vi "drawTempRectangle.vi"(0 "reference":refnum<class "Graphics.lvclass">, 1 "rectangle":T1 {"height" format="%.2f"; "width" format="%.2f"; "y" format="%.2f"; "x" format="%.2f"}, 2 "lineWidth(1)":dbl=1.0 format="%.2f", 3 "color(if not used=default color)":u32=33554432 format="%.0x", 4 "fill?(F)":bool, 5 "error in (no error)":errorcluster, 6 "Rectangles":T1[](array[typedef]) {"height" format="%.2f"; "width" format="%.2f"; "y" format="%.2f"; "x" format="%.2f"}, 7 "readFromMaster(True)":bool=TRUE) -> (14 "reference out":refnum<class "Graphics.lvclass">, 16 "picture":picture, 19 "error out":errorcluster)   [LabVIEW 2020, in "Graphics.lvclass"]
doc: "Draws a rectangle"
uses:
  <resource>/Framework/Providers/Open_GDS/UML/Graphics_class/Graphics.lvclass
  <resource>/Framework/Providers/Open_GDS/UML/General/Rectangle/Rectangle Rectangle2D.ctl
panel:
  # "Always set\nVI Server class\nto current VI. Do not\nconnect this control\nto the connector pane.\n(Tip!: Just drag\nand drop the icon\ninto the refnum)"
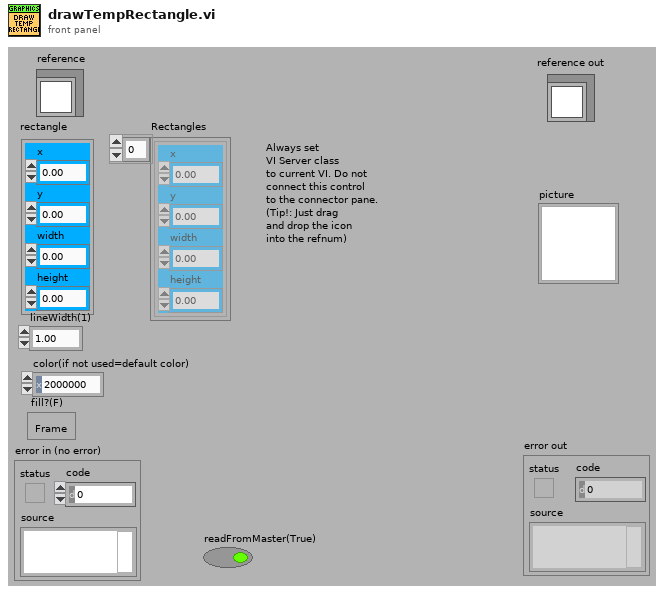
[diagram p1: front panel]
types:
  T1 = typedef "Rectangle Rectangle2D.ctl" = cluster{"x":dbl, "y":dbl, "width":dbl, "height":dbl}
  T2 = typedef "Graphics.lvclass/ObjectAttributes.ctl" = cluster{"drawColor":u32, "backgroundColor":u32, "font":T3, "fontType":T4, "picture":picture, "stroke":T5, "scaleX":dbl, "scaleY":dbl, "screenRef":refnum<vi>, "offsetX":dbl, "offsetY":dbl}
  T3 = typedef "Graphics.lvclass/FontType.ctl" = cluster{"Font Name:":string, "Size":i16, "Strikeout?":bool, "Italic?":bool, "Underline?":bool, "Outline?":bool, "Shadow?":bool, "Bold?":bool}
  T4 = typedef "Graphics.lvclass/LvFontType.ctl" = enum16{"User-specified Font", "Application Font", "System Font", "Dialog Font"}
  T5 = typedef "Graphics.lvclass/StrokeType.ctl" = enum16{"USE_DEFAULT", "SOLID", "DOTTED"}
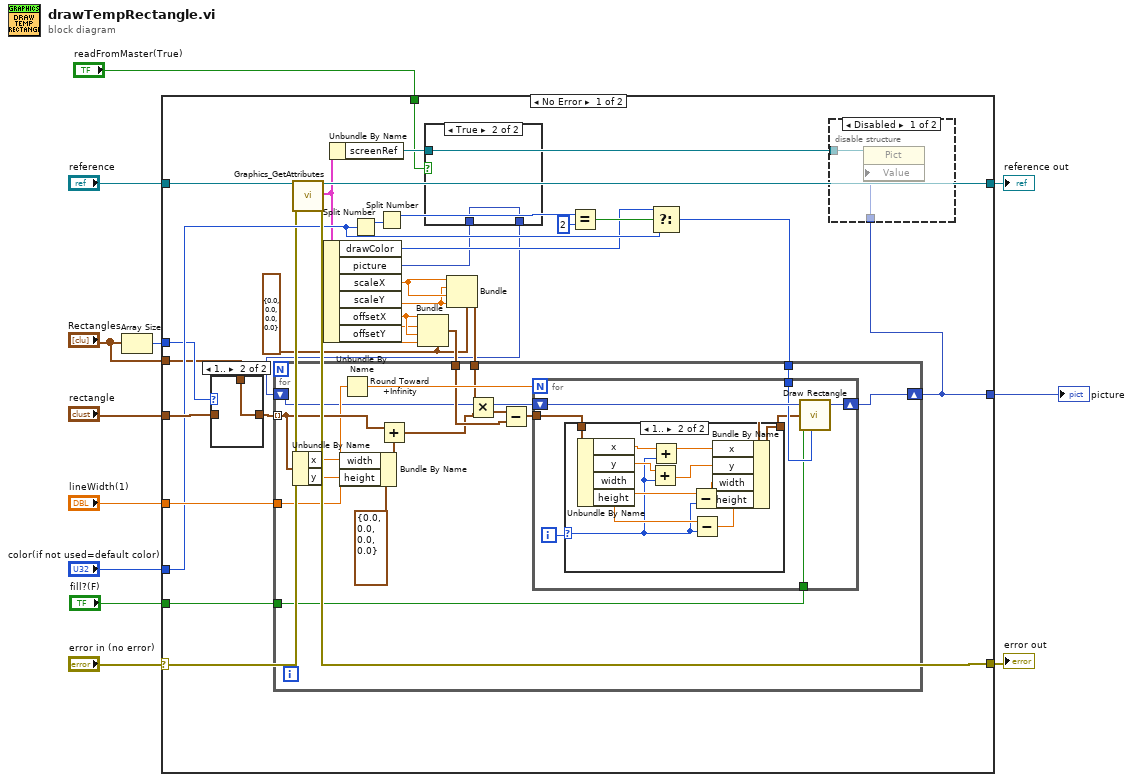
[diagram p0: block diagram]
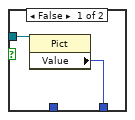
[diagram p3: hidden frame]
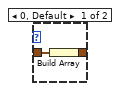
[diagram p4: hidden frame]
diagram:
  n1 = Array Size(array="Rectangles") -> (size(s)=w4:i32)
  n2 = case shown="No Error" "error in (no error)" {
    selector: "error in (no error)" -> [w35 w86]
    tunnel: "reference" -> [w42 w87]
    tunnel: [w41 w86] -> w11
    tunnel: [w40 w87] -> w10
    tunnel: "rectangle" -> [w39 _]
    tunnel: "lineWidth(1)" -> [w38 _]
    tunnel: "color(if not used=default color)" -> [w37 _]
    tunnel: "fill?(F)" -> [w36 _]
    tunnel: w4 -> [w18 _]
    tunnel: "Rectangles" -> [w17 _]
    tunnel: "readFromMaster(True)" -> [w14 _]
    tunnel: [w13 _] -> w1
    frame No Error {
      w20 = T1 {"x"=0.0, "y"=0.0, "width"=0.0, "height"=0.0} ("rectangle")
      n3 = case shown="1.." w18 {
        tunnel: w39 -> [w49 _]
        tunnel: [w48 w50] -> w19
        tunnel: w17 -> [_ w50]
        frame 0, Default {
          n4 = Build Array(w49) -> (w48:T1[])
        }
        frame 1.. {
        }
      }
      n5 = call <resource>:"Graphics_GetAttributes.vi"("reference in"=w42, "error in (no error)"=w35) -> ("reference out"=w40:refnum<class "Graphics.lvclass">, "Data"=w15:T2, "error out"=w41:errorcluster)  [unwired: 1 in, 14 out]
      n6 = Unbundle By Name(w15) -> ("drawColor"=w30:u32, "picture"=w21:picture, "scaleX"=w27:dbl, "scaleY"=w26:dbl, "offsetX"=w25:dbl, "offsetY"=w24:dbl)
      n7 = Unbundle By Name(w15) -> ("screenRef"=w22:refnum<vi>)
      n8 = Split Number(x=w37) -> (hi(x)=w34:u16)  [unwired: 1 out]
      n9 = Split Number(x=w34) -> (hi(x)=w33:u8)  [unwired: 1 out]
      n10 = Bundle(cluster=w20, "x"=w25, "y"=w24, "width"=w25, "height"=w24) -> (w23:T1)
      n11 = case shown="True" w14 {
        tunnel: w22 -> [w46 _]
        tunnel: w21 -> [_ w47]
        tunnel: [w45 w47] -> w16
        frame False {
          n12 = property class="Pict"(reference=w46) -> ("Value"=w45:picture)  [unwired: 1 in, 2 out]
        }
        frame True {
        }
      }
      n13 = Bundle(cluster=w20, "x"=w27, "y"=w26, "width"=w27, "height"=w26) -> (w28:T1)
      n14 = Equal?(x=w33, y=u8 2) -> (x = y?=w31:bool)
      n15 = Select(t=w30, s=w31, f=w37) -> (s? t:f=w29:u32)
      n16 = for {
        tunnel: w19 -> [w66] mode=indexing
        tunnel: w38 -> [w65]
        tunnel: w36 -> [w64]
        tunnel: w29 -> [w62]
        tunnel: w28 -> [w61]
        tunnel: w23 -> [w54]
        shift-right: [w52] -> w13
        shift-left: w16 -> [w51]
        n17 = Unbundle By Name(w66) -> ("x"=w59:dbl, "y"=w58:dbl)
        n18 = Bundle By Name(cluster=T1 {"x"=0.0, "y"=0.0, "width"=0.0, "height"=0.0} ("x"), "width"=w59, "height"=w58) -> (w57:T1)
        n19 = Round Toward +Infinity(x=w65) -> (ceil(x): smallest int >= x=w63:dbl)
        n20 = Add(x=w66, y=w57) -> (x+y=w53:T1)
        n21 = Multiply(x=w61, y=w53) -> (x*y=w56:T1)
        n22 = Subtract(x=w56, y=w54) -> (x-y=w55:T1)
        n23 = for {
          N: w63 -> [_]
          tunnel: w55 -> [w69]
          tunnel: w62 -> [w72]
          shift-right: [w71] -> w52
          shift-left: w51 -> [w73]
          tunnel: w64 -> [w67]
          i -> [w68]
          n24 = case shown="1.." w68 {
            selector: w68 -> [_ w75]
            tunnel: [w74 w77] -> w70
            tunnel: w69 -> [w74 w76]
            frame 0, Default {
            }
            frame 1.. {
              n25 = Unbundle By Name(w76) -> ("x"=w85:dbl, "y"=w84:dbl, "width"=w83:dbl, "height"=w82:dbl)
              n26 = Add(x=w84, y=w75) -> (x+y=w80:dbl)
              n27 = Add(x=w85, y=w75) -> (x+y=w81:dbl)
              n28 = Subtract(x=w83, y=w75) -> (x-y=w79:dbl)
              n29 = Subtract(x=w82, y=w75) -> (x-y=w78:dbl)
              n30 = Bundle By Name(cluster=w76, "x"=w81, "y"=w80, "width"=w79, "height"=w78) -> (w77:T1)
            }
          }
          n31 = call <vilib>:"Draw Rectangle.vi"("picture"=w73, "rect"=w70, "fill?(F)"=w67, "color(black)"=w72) -> ("new picture"=w71:picture)  [unwired: 5 in]
        }
      }
      n32 = disable-structure shown="Disabled" {
        disable-tunnel: w22 -> [w44 _]
        disable-tunnel: w13 -> [w43 _]
        frame Disabled {
          n33 = property class="Pict"(reference=w44, "Value"=w43) -> ()  [unwired: 1 in, 2 out]
        }
        frame Enabled {
        }
      }
    }
    frame Error {
    }
  }
  "reference out" <- w10
  "error out" <- w11
  "picture" <- w1
